vi "Test testCoordinator API.vi"() -> ()   [LabVIEW 2026]
doc: "testCoordinator API Tester."
uses:
  <vilib>/Utility/error.llb/DialogType.ctl
  215ddbd9-6c16-4e6c-8331-101f4cb2082d.vi
  modules/coordinator/src/Libraries/Core/global.vi
  <vilib>/Utility/error.llb/Search and Replace Pattern (string).vi
  <vilib>/JDP Science/JSONtext/Variant to JSON Text.vi
  <vilib>/JDP Science/JSONtext/LVClass Serializer/JSONtext LVClass Serializer.lvclass
  testCoordinator.lvlib
panel:
  out "Test Scope":string
  out "Test Procedure File Name":string
  in  "Multicolumn Listbox":i32(listbox)=-1
  in  "Begin Test Execution":bool
  in  "Manual Tests Folder":path=path "C:/Users/Public/Documents/svelderrainruiz/Manual Tests"
  in  "Set Manual Tests Folder Location":bool
  out "last error":errorcluster
  in  "Show Diagram on Init":bool
  in  "wait for reply":bool=TRUE
  in  "Show Block Diagram":bool
  in  "X":dbl=1.0
  out "Reply Payload":dbl
  in  "Stop Module":bool
  in  "Start Module":bool
  out "Do Something Count":i32
  in  "Test Do Something Else and Wait for Reply":bool
  in  "Hide Module Panel":bool
  in  "Show Module Panel":bool
  in  "Test Do Something Else":bool
  in  "Test Do Something":bool
  out "Status":string
  out "Module Running?":bool
  # "- Create a VI that tests if an .md file is compatible."
  # "This VI tests the API for the Module."
  # "Start Manual Test"
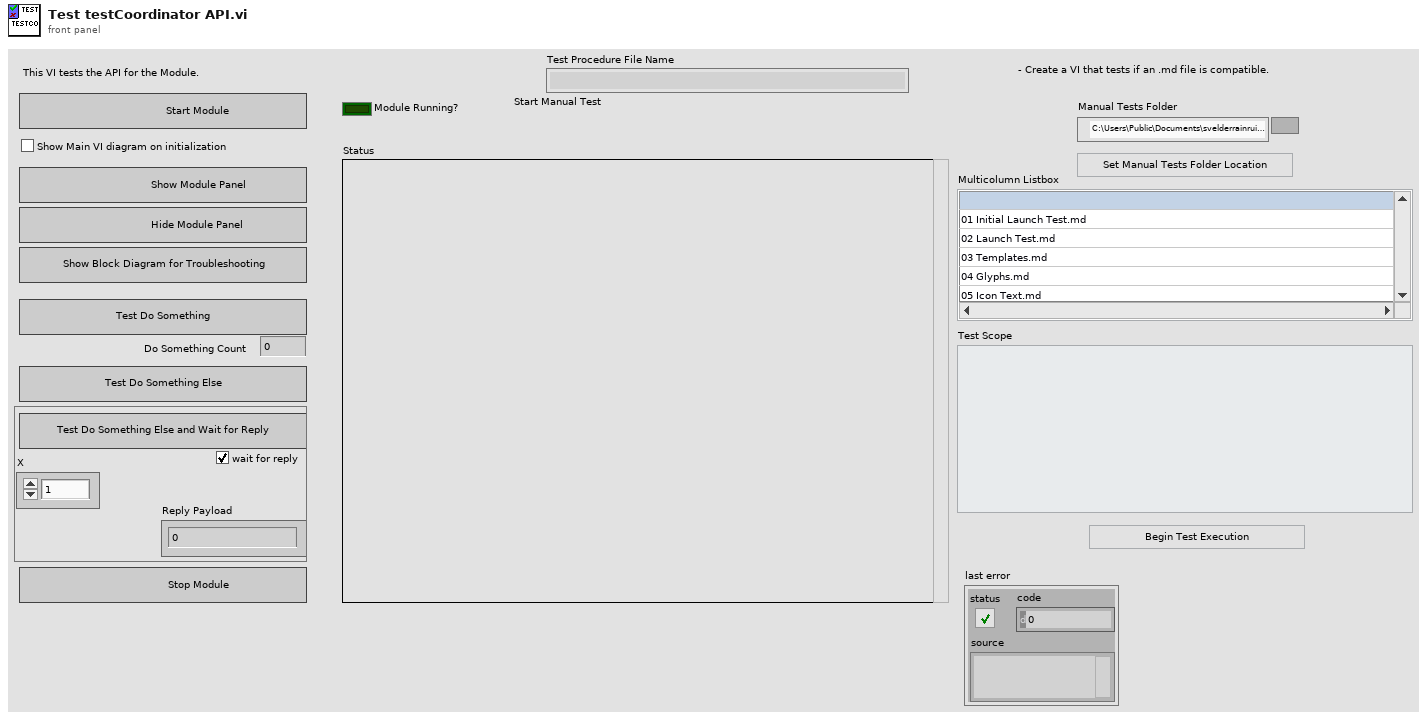
[diagram p1: front panel]
types:
  T1 = typedef "testCoordinator.lvlib/Broadcast Events--cluster.ctl" = cluster{"Module Did Init":refnum<user-event>, "Status Updated":refnum<user-event>, "Error Reported":refnum<user-event>, "Did Something":refnum<user-event>, "Module Did Stop":refnum<user-event>, "Update Module Execution Status":refnum<user-event>, "Broadcast Available Tests":refnum<user-event>, "Refresh Test Procedure Indicator":refnum<user-event>, "Refresh Section Indicator":refnum<user-event>, "Refresh Instruction Indicator":refnum<user-event>, "Broadcast Test Scope":refnum<user-event>, "Broadcast Actual Test Procedure Section":refnum<user-event>}
  T2 = typedef "DialogType.ctl" = u16
  T3 = typedef "testCoordinator.lvlib/Do Something Else and Wait (Reply Payload)--cluster.ctl" = cluster{"Value":dbl, "error":errorcluster}
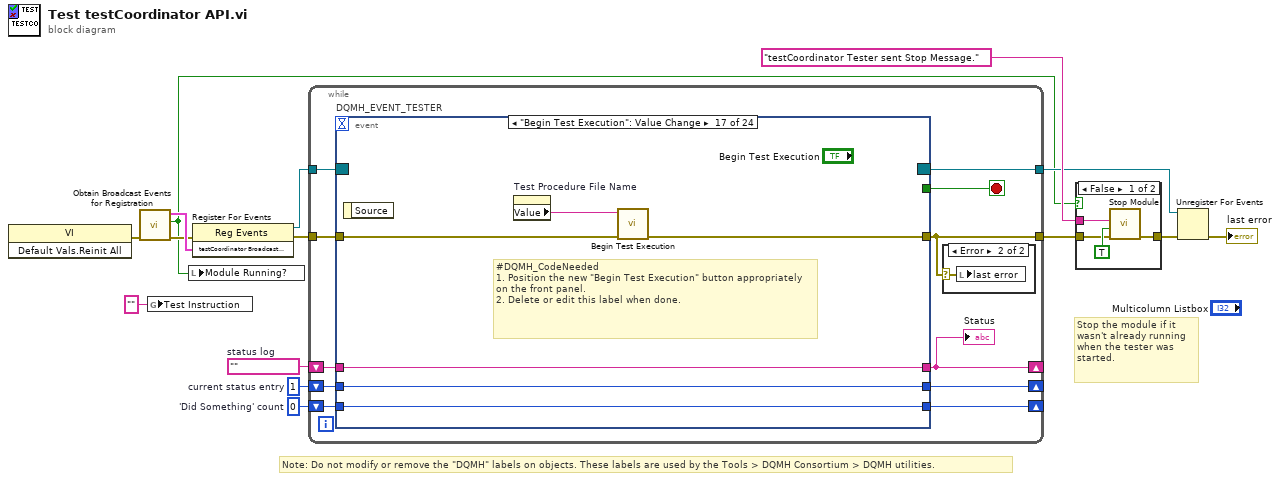
[diagram p0: block diagram]
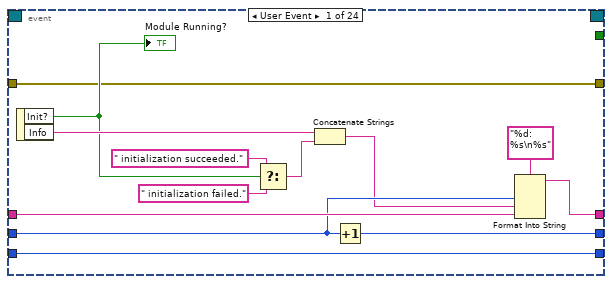
[diagram p4: hidden frame]
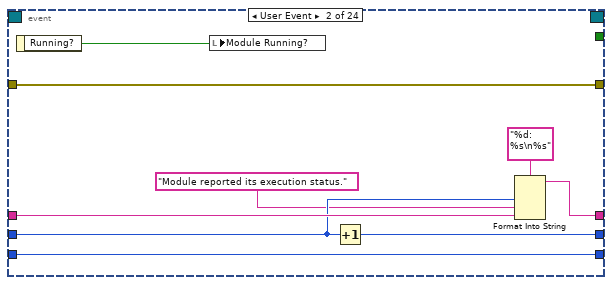
[diagram p5: hidden frame]
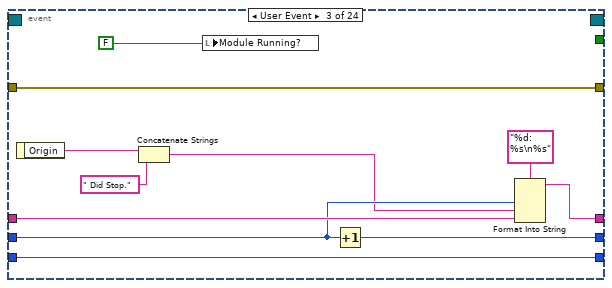
[diagram p6: hidden frame]
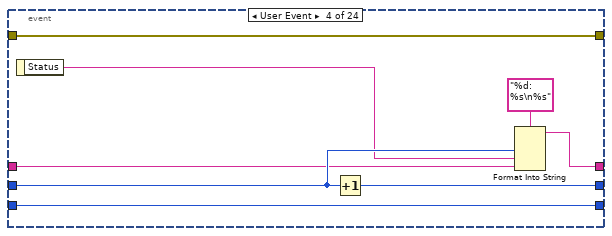
[diagram p7: hidden frame]
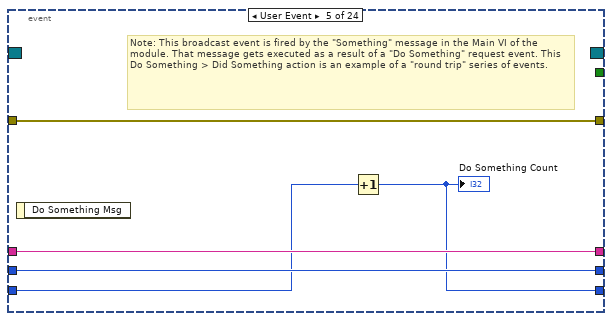
[diagram p8: hidden frame]
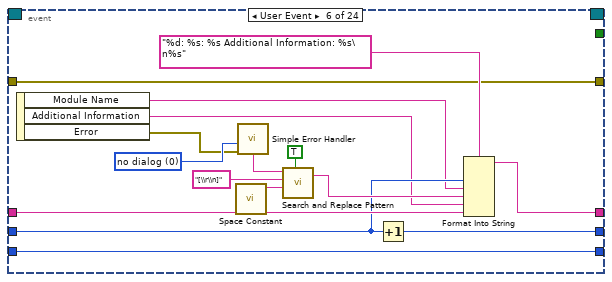
[diagram p9: hidden frame]
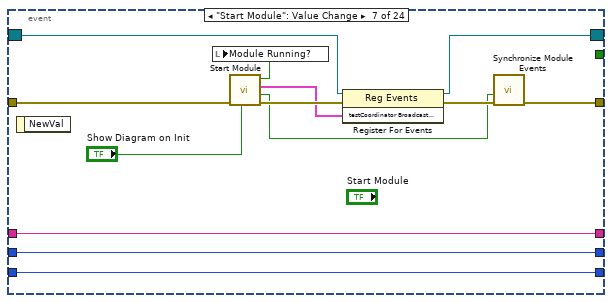
[diagram p10: hidden frame]
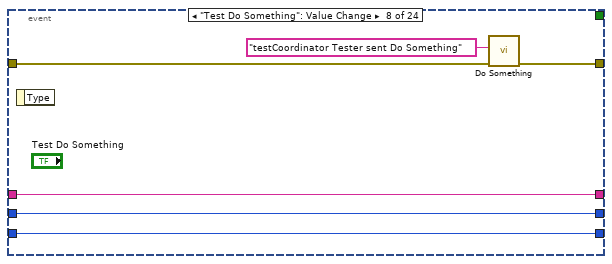
[diagram p11: hidden frame]
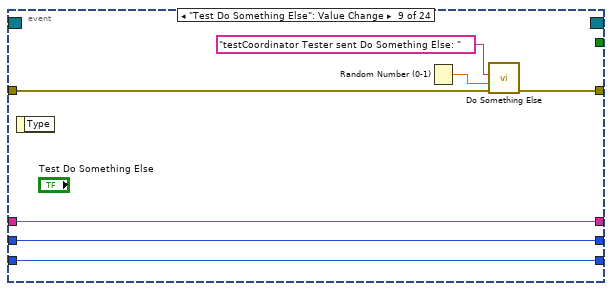
[diagram p12: hidden frame]
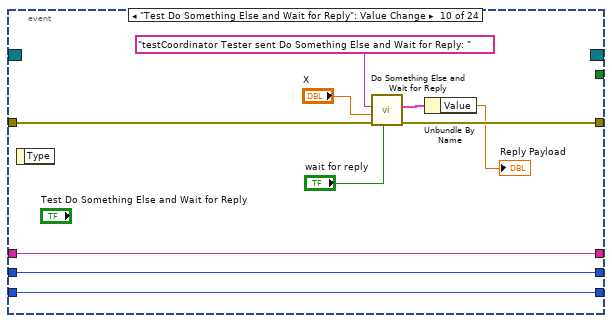
[diagram p13: hidden frame]
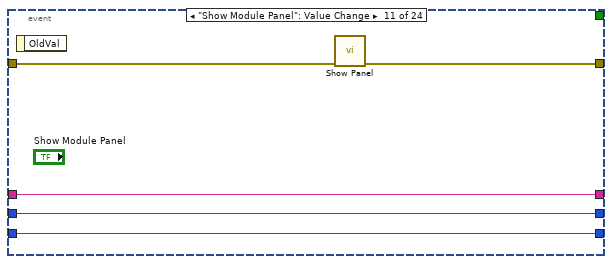
[diagram p14: hidden frame]
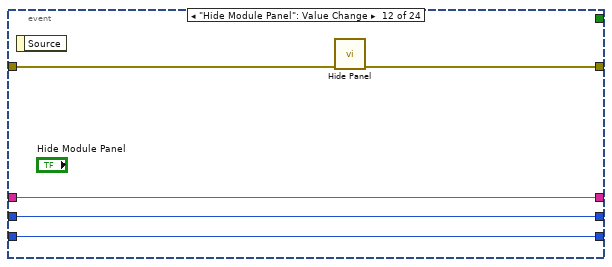
[diagram p15: hidden frame]
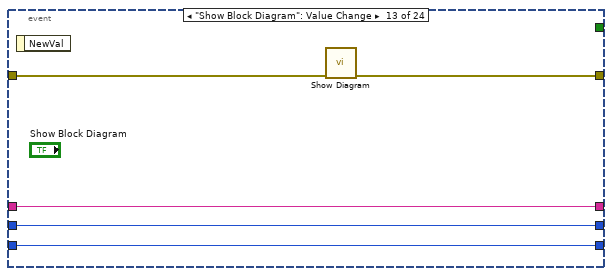
[diagram p16: hidden frame]
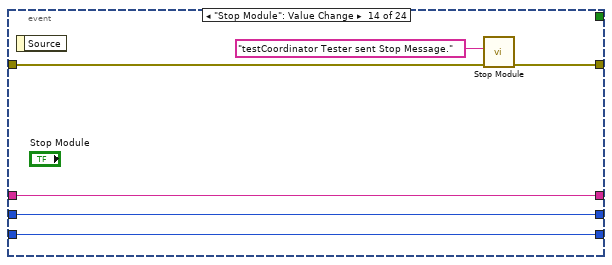
[diagram p17: hidden frame]
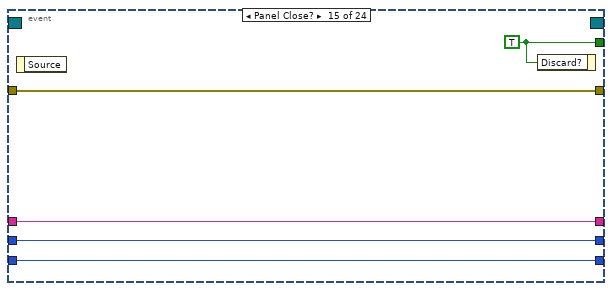
[diagram p18: hidden frame]
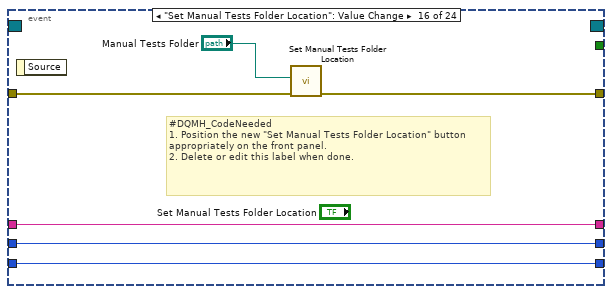
[diagram p19: hidden frame]
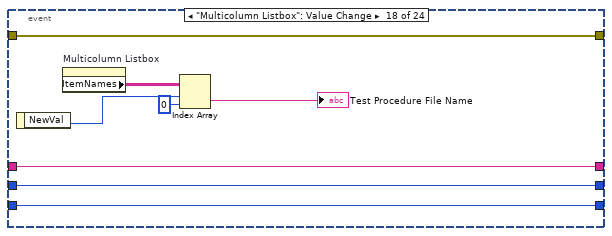
[diagram p20: hidden frame]
diagram:
  w11 = 0  # 'Did Something' count
  w12 = 1  # current status entry
  w13 = ""  # status log
  # "Stop the module if it wasn't already running when the tester was started."
  # "Note: Do not modify or remove the \"DQMH\" labels on objects. These labels are used by the Tools > DQMH Consortium > DQMH utilities."
  n1 = invoke class="VI" method="Default Vals.Reinit All"() -> (error out=w6:errorcluster)  [unwired: 3 in, 2 out]
  n2 = call "Obtain Broadcast Events for Registration.vi"("error in"=w6) -> ("error out"=w5:errorcluster, "Already running?"=w4:bool, "testCoordinator Broadcast Events"=w9:T1)  [unwired: 8 in]
  n3 = global write "global.vi" "Test Instruction"("" ("Test Instruction")) -> ()
  n4 = local write "Module Running?"(w4) -> ()
  n5 = register-events(error in=w5, w9) -> (reference out=w8:refnum<event-registration>, error out=w10:errorcluster)  [unwired: 1 in]
  n6 = while {
    tunnel: w8 -> [w26]
    tunnel: [w16] -> w3
    shift-right: [w22] -> _
    shift-left: w13 -> [w24]
    shift-right: [w23] -> _
    shift-left: w12 -> [w25]
    shift-right: [w20] -> _
    shift-left: w11 -> [w21]
    tunnel: w10 -> [w19]
    tunnel: [w18] -> w7
    stop <- w17 stop-if-true
    n7 = event "DQMH_EVENT_TESTER" shown="[16] \"Begin Test Execution\": Value Change" {
      selector: w26 -> [_ _ _ _ _ _ w95 _ _ _ _ _ _ _ _ _ _ _ _ _ _ _ _ _]
      dyn-events: [_ _ _ _ _ _ w94 _ _ _ _ _ _ _ _ _ _ _ _ _ _ _ _ _] -> w18
      timeout: _ -> [_ _ _ _ _ _ _ _ _ _ _ _ _ _ _ _ _ _ _ _ _ _ _ _]
      tunnel: [_ _ _ _ _ _ _ _ _ _ _ _ _ _ w151 _ _ _ _ _ _ _ _ _] -> w17
      tunnel: [w28 w42 w50 w61 w69 w77 w90 w108 w115 w125 w130 w135 w136 w143 w147 w153 w159 w165 w182 w192 w202 w212 w222 w232] -> w16
      tunnel: w25 -> [w38 w47 w58 w65 w72 w80 w99 w105 w111 w122 w128 w133 w138 w145 w149 w155 w161 w170 w178 w188 w198 w208 w218 w228]
      tunnel: w24 -> [w39 w48 w59 w64 w73 w81 w100 w106 w112 w123 w129 w134 w139 w146 w150 w156 w162 w171 w180 w190 w200 w210 w220 w230]
      tunnel: [w36 w45 w56 w66 w73 w79 w100 w106 w112 w123 w129 w134 w139 w146 w150 w156 w162 w171 w179 w189 w199 w209 w219 w229] -> w22
      tunnel: [w37 w46 w57 w68 w72 w78 w99 w105 w111 w122 w128 w133 w138 w145 w149 w155 w161 w170 w177 w187 w197 w207 w217 w227] -> w23
      tunnel: w21 -> [w33 w43 w52 w62 w71 w89 w98 w104 w110 w121 w127 w132 w137 w144 w148 w154 w160 w169 w181 w191 w201 w211 w221 w231]
      tunnel: [w33 w43 w52 w62 w70 w89 w98 w104 w110 w121 w127 w132 w137 w144 w148 w154 w160 w169 w181 w191 w201 w211 w221 w231] -> w20
      tunnel: w19 -> [w28 w42 w50 w61 w69 w77 w93 w103 w109 w118 w126 w131 w140 w141 w147 w157 w163 w165 w182 w192 w202 w212 w222 w232]
      event User Event {
        n8 = event-data() -> ("Init?"=w32:bool, "Info"=w35:string)  [unwired: 1 in]
        "Module Running?" <- w32
        n9 = Select(t=" initialization succeeded.", s=w32, f=" initialization failed.") -> (s? t:f=w29:string)
        n10 = Concatenate Strings(w35, w29) -> (w34:string)
        n11 = Increment(x=w38) -> (x+1=w37:i32)
        n12 = Format Into String(format string="%d: %s\n%s", w38, w34, w39) -> (resulting string=w36:string)  [unwired: 2 in, 1 out]
      }
      event User Event {
        n13 = event-data() -> ("Running?"=w41:bool)  [unwired: 1 in]
        n14 = local write "Module Running?"(w41) -> ()
        n15 = Increment(x=w47) -> (x+1=w46:i32)
        n16 = Format Into String(format string="%d: %s\n%s", w47, "Module reported its execution status.", w48) -> (resulting string=w45:string)  [unwired: 2 in, 1 out]
      }
      event User Event {
        n17 = event-data() -> ("Origin"=w55:string)  [unwired: 1 in]
        n18 = Concatenate Strings(w55, " Did Stop.") -> (w54:string)
        n19 = local write "Module Running?"(FALSE ("Module Did Init?")) -> ()
        n20 = Increment(x=w58) -> (x+1=w57:i32)
        n21 = Format Into String(format string="%d: %s\n%s", w58, w54, w59) -> (resulting string=w56:string)  [unwired: 2 in, 1 out]
      }
      event User Event {
        n22 = event-data() -> ("Status"=w63:string)  [unwired: 1 in]
        n23 = Increment(x=w65) -> (x+1=w68:i32)
        n24 = Format Into String(format string="%d: %s\n%s", w65, w63, w64) -> (resulting string=w66:string)  [unwired: 2 in, 1 out]
      }
      event User Event {
        # "Note: This broadcast event is fired by the \"Something\" message in the Main VI of the module. That message gets executed as a result of a \"Do Something\" request event. This Do Something > Did Something action is an example of a \"round trip\" series of events."
        n25 = event-data() -> ()  [unwired: 1 in, 1 out]
        n26 = Increment(x=w71) -> (x+1=w70:i32)
        "Do Something Count" <- w70
      }
      event User Event {
        w82 = T2 0 items=["no dialog", "OK message", "continue or stop message", "OK message + warnings", "continue/stop + warnings"] ("type of dialog (OK msg:1)")
        n27 = event-data() -> ("Module Name"=w76:string, "Additional Information"=w75:string, "Error"=w74:errorcluster)  [unwired: 1 in]
        n28 = call <vilib>:"Space Constant.vi"() -> ("String"=w86:string)
        n29 = call <vilib>:"Simple Error Handler.vi"("type of dialog (OK msg:1)"=w82, "error in (no error)"=w74) -> ("message"=w83:string)  [unwired: 3 in, 4 out]
        n30 = call-poly <vilib>:"Search and Replace Pattern.vi"("string"=w83, "regular expression (\"\")"="[\\r\\n]" ("regular expression (\"\")"), "replace string (\"\")"=w86, "replace all? (F)"=TRUE ("replace all CR/LF with spaces")) -> ("result string"=w84:string)  [unwired: 1 in, 1 out]
        n31 = Increment(x=w80) -> (x+1=w78:i32)
        n32 = Format Into String(format string="%d: %s: %s Additional Information: %s\n%s", w80, w76, w84, w75, w81) -> (resulting string=w79:string)  [unwired: 2 in, 1 out]
      }
      event "Start Module": Value Change {
        n33 = event-data() -> ()  [unwired: 1 in, 1 out]
        n34 = call "Start Module.vi"("Show Main VI Diagram on Init (F)"="Show Diagram on Init", "error in"=w93) -> ("error out"=w101:errorcluster, "Wait for Event Sync?"=w97:bool, "testCoordinator Broadcast Events"=w96:T1, "Module Was Already Running?"=w92:bool)  [unwired: 5 in, 1 out]
        n35 = local write "Module Running?"(w92) -> ()
        n36 = register-events(reference=w95, error in=w101, w96) -> (reference out=w94:refnum<event-registration>, error out=w102:errorcluster)
        n37 = call "Synchronize Module Events.vi"("error in"=w102, "Wait for Event Sync?"=w97) -> ("error out"=w90:errorcluster)  [unwired: 9 in]
      }
      event "Test Do Something": Value Change {
        n38 = event-data() -> ()  [unwired: 1 in, 1 out]
        n39 = call "Do Something.vi"("error in"=w103, "Do Something Message"="testCoordinator Tester sent Do Something") -> ("error out"=w108:errorcluster)  [unwired: 9 in]
      }
      event "Test Do Something Else": Value Change {
        n40 = event-data() -> ()  [unwired: 1 in, 1 out]
        n41 = Random Number (0-1)() -> (number: 0 to 1=w113:dbl)
        n42 = call "Do Something Else.vi"("error in"=w109, "X"=w113, "Do Something Else Message"="testCoordinator Tester sent Do Something Else: " ("Do Something Message")) -> ("error out"=w115:errorcluster)  [unwired: 8 in]
      }
      event "Test Do Something Else and Wait for Reply": Value Change {
        n43 = event-data() -> ()  [unwired: 1 in, 1 out]
        n44 = call "Do Something Else and Wait for Reply.vi"("wait for reply (T)"="wait for reply", "error in"=w118, "X"="X", "Do Something Else Message"="testCoordinator Tester sent Do Something Else and Wait for Reply: " ("Do Something Message")) -> ("error out"=w125:errorcluster, "Reply Payload"=w120:T3)  [unwired: 5 in, 1 out]
        n45 = Unbundle By Name(w120) -> ("Value"=→"Reply Payload":dbl)
      }
      event "Show Module Panel": Value Change {
        n46 = event-data() -> ()  [unwired: 1 in, 1 out]
        n47 = call "Show Panel.vi"("error in"=w126) -> ("error out"=w130:errorcluster)  [unwired: 10 in]
      }
      event "Hide Module Panel": Value Change {
        n48 = event-data() -> ()  [unwired: 1 in, 1 out]
        n49 = call "Hide Panel.vi"("error in"=w131) -> ("error out"=w135:errorcluster)  [unwired: 10 in]
      }
      event "Show Block Diagram": Value Change {
        n50 = event-data() -> ()  [unwired: 1 in, 1 out]
        n51 = call "Show Diagram.vi"("error in"=w140) -> ("error out"=w136:errorcluster)  [unwired: 10 in]
      }
      event "Stop Module": Value Change {
        n52 = event-data() -> ()  [unwired: 1 in, 1 out]
        n53 = call "Stop Module.vi"("error in"=w141, "Origin"="testCoordinator Tester sent Stop Message.") -> ("error out"=w143:errorcluster)  [unwired: 9 in]
      }
      event Panel Close? {
        w151 = TRUE ("Discard?")
        n54 = event-data() -> ()  [unwired: 1 in, 1 out]
        n55 = event-data("Discard?"=w151) -> ()  [unwired: 1 in, 1 out]
      }
      event "Set Manual Tests Folder Location": Value Change {
        # "#DQMH_CodeNeeded\n1. Position the new \"Set Manual Tests Folder Location\" button appropriately on the front panel.\n2. Delete or edit this label when done."
        n56 = event-data() -> ()  [unwired: 1 in, 1 out]
        n57 = call "Set Manual Tests Folder Location.vi"("error in"=w157, "Manual Tests Folder"="Manual Tests Folder") -> ("error out"=w153:errorcluster)  [unwired: 7 in, 2 out]
      }
      event "Begin Test Execution": Value Change {
        # "#DQMH_CodeNeeded\n1. Position the new \"Begin Test Execution\" button appropriately on the front panel.\n2. Delete or edit this label when done."
        n58 = event-data() -> ()  [unwired: 1 in, 1 out]
        n59 = property on="Test Procedure File Name" class="Str"() -> ("Value"=w158:string)  [unwired: 2 in, 2 out]
        n60 = call "Begin Test Execution.vi"("error in"=w163, "Test Procedure"=w158) -> ("error out"=w159:errorcluster)  [unwired: 9 in]
      }
      event "Multicolumn Listbox": Value Change {
        n61 = event-data() -> ("NewVal"=w167:i32)  [unwired: 1 in]
        n62 = property on="Multicolumn Listbox" class="MCListbox (strict)"() -> ("ItemNames"=w168:string[][])  [unwired: 2 in, 2 out]
        n63 = Index Array(array=w168, index (row)=w167, index (col)=0 ("disabled index (col)")) -> (element=→"Test Procedure File Name":string)
      }
      event User Event {
        # "#DQMH_CodeNeeded Replace this format string with a meaningful value for this broadcast, then wire broadcast data from the Event Data Node to the input(s) of the Format Into String function."
        # "#DQMH_CodeNeeded\n1. Process the event data sent by the \"Broadcast Available Tests\" broadcast event.\n2. Delete or edit this label when done."
        n64 = event-data() -> ("Available Tests"=w173:string[][])  [unwired: 1 in]
        n65 = property on="Multicolumn Listbox" class="MCListbox (strict)"("ItemNames"=w173) -> ()  [unwired: 2 in, 2 out]
        n66 = call "To JSON Text.vim"("Anything"=w173) -> ("<JSON>"=w172:string)  [unwired: 9 in, 1 out]
        n67 = Format Into String(format string="Response Received - %s", w172) -> (resulting string=w174:string)  [unwired: 2 in, 1 out]
        n68 = Increment(x=w178) -> (x+1=w177:i32)
        n69 = Format Into String(format string="%d: %s\n%s", w178, w174, w180) -> (resulting string=w179:string)  [unwired: 2 in, 1 out]
      }
      event User Event {
        # "#DQMH_CodeNeeded Replace this format string with a meaningful value for this broadcast, then wire broadcast data from the Event Data Node to the input(s) of the Format Into String function."
        # "#DQMH_CodeNeeded\n1. Process the event data sent by the \"Refresh Test Procedure Indicator\" broadcast event.\n2. Delete or edit this label when done."
        n70 = event-data() -> ("Test Procedure"=w183:string)  [unwired: 1 in, 4 out]
        n71 = Format Into String(format string="Response Received - %s", w183) -> (resulting string=w184:string)  [unwired: 2 in, 1 out]
        n72 = Increment(x=w188) -> (x+1=w187:i32)
        n73 = Format Into String(format string="%d: %s\n%s", w188, w184, w190) -> (resulting string=w189:string)  [unwired: 2 in, 1 out]
      }
      event User Event {
        # "#DQMH_CodeNeeded Replace this format string with a meaningful value for this broadcast, then wire broadcast data from the Event Data Node to the input(s) of the Format Into String function."
        # "#DQMH_CodeNeeded\n1. Process the event data sent by the \"Refresh Section Indicator\" broadcast event.\n2. Delete or edit this label when done."
        n74 = event-data() -> ("Section"=w193:string)  [unwired: 1 in, 4 out]
        n75 = Format Into String(format string="Response Received - %s", w193) -> (resulting string=w194:string)  [unwired: 2 in, 1 out]
        n76 = Increment(x=w198) -> (x+1=w197:i32)
        n77 = Format Into String(format string="%d: %s\n%s", w198, w194, w200) -> (resulting string=w199:string)  [unwired: 2 in, 1 out]
      }
      event User Event {
        n78 = event-data() -> ("Instruction"=w203:string)  [unwired: 1 in]
        n79 = Format Into String(format string="Response Received - %s", w203) -> (resulting string=w204:string)  [unwired: 2 in, 1 out]
        n80 = Increment(x=w208) -> (x+1=w207:i32)
        n81 = Format Into String(format string="%d: %s\n%s", w208, w204, w210) -> (resulting string=w209:string)  [unwired: 2 in, 1 out]
      }
      event User Event {
        # "#DQMH_CodeNeeded Replace this format string with a meaningful value for this broadcast, then wire broadcast data from the Event Data Node to the input(s) of the Format Into String function."
        # "#DQMH_CodeNeeded\n1. Process the event data sent by the \"Broadcast Test Scope\" broadcast event.\n2. Delete or edit this label when done."
        n82 = event-data() -> ("Test Scope"=w213:string)  [unwired: 1 in]
        "Test Scope" <- w213
        n83 = Format Into String(format string="Response Received - %s", w213) -> (resulting string=w214:string)  [unwired: 2 in, 1 out]
        n84 = Increment(x=w218) -> (x+1=w217:i32)
        n85 = Format Into String(format string="%d: %s\n%s", w218, w214, w220) -> (resulting string=w219:string)  [unwired: 2 in, 1 out]
      }
      event User Event {
        # "#DQMH_CodeNeeded Replace this format string with a meaningful value for this broadcast, then wire broadcast data from the Event Data Node to the input(s) of the Format Into String function."
        # "#DQMH_CodeNeeded\n1. Process the event data sent by the \"Broadcast Actual Test Procedure Section\" broadcast event.\n2. Delete or edit this label when done."
        n86 = event-data() -> ("Section"=w223:string)  [unwired: 1 in, 4 out]
        n87 = Format Into String(format string="Response Received - %s", w223) -> (resulting string=w224:string)  [unwired: 2 in, 1 out]
        n88 = Increment(x=w228) -> (x+1=w227:i32)
        n89 = Format Into String(format string="%d: %s\n%s", w228, w224, w230) -> (resulting string=w229:string)  [unwired: 2 in, 1 out]
      }
    }
    "Status" <- w22
    n90 = case shown="Error" w16 {
      selector: w16 -> [_ w27]
      frame No Error {
      }
      frame Error {
        n91 = local write "last error"(w27) -> ()
      }
    }
  }
  n92 = case shown="False" w4 {
    tunnel: [w236 w237] -> w15
    tunnel: "testCoordinator Tester sent Stop Message." ("Origin") -> [w235 _]
    tunnel: w3 -> [w233 w237]
    frame False {
      n93 = call "Stop Module.vi"("error in"=w233, "Wait for Module to Stop? (F)"=TRUE ("Wait for Module to stop?"), "Origin"=w235) -> ("error out"=w236:errorcluster)  [unwired: 8 in]
    }
    frame True {
    }
  }
  n94 = Unregister For Events(event registration refnum=w7, error in=w15) -> (error out=→"last error":errorcluster)
